vi "TDMS_EnsureFile.vi"(8 "error in (no error)":errorcluster, 11 "Logger_state":T1={"ref TDMS"=refnum, "File Path"=path "", "counter"=0, "Folder tmp"=path "/home/lvuser/lab9data/tmp", "folder ready"=path "/home/lvuser/lab9data/ready"}) -> (0 "error out":errorcluster, 3 "state out":T1)   [LabVIEW 2025]
uses:
  Logger_State.ctl
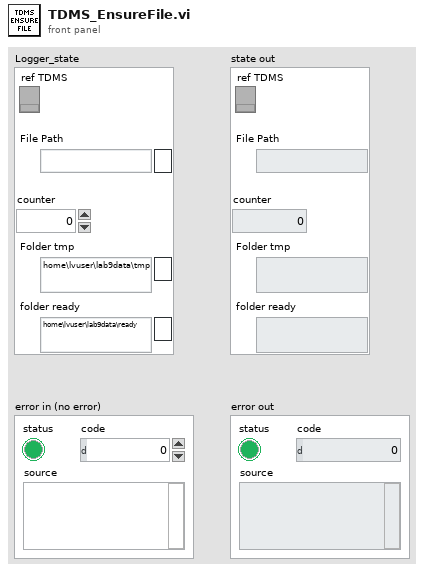
[diagram p1: front panel]
types:
  T1 = typedef "Logger_State.ctl" = cluster{"ref TDMS":refnum<k34>, "File Path":path, "counter":i32, "Folder tmp":path, "folder ready":path}
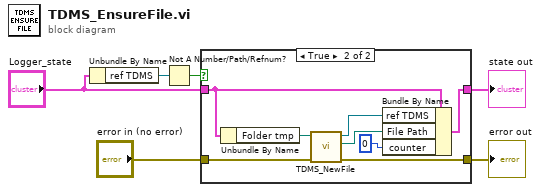
[diagram p0: block diagram]
diagram:
  n1 = Unbundle By Name("Logger_state") -> ("ref TDMS"=w1:refnum<k34>)
  n2 = Not A Number/Path/Refnum?(number/path/refnum=w1) -> (NaN/Path/Refnum?=w2:bool)
  n3 = case shown="True" w2 {
    tunnel: "Logger_state" -> [w7 w14]
    tunnel: "error in (no error)" -> [w8 w9]
    tunnel: [w8 w15] -> w5
    tunnel: [w7 w10] -> w6
    frame False {
    }
    frame True {
      n4 = Unbundle By Name(w14) -> ("Folder tmp"=w16:path)
      n5 = call "TDMS_NewFile.vi"("error in (no error)"=w9, "Folder tmp"=w16) -> ("error out"=w15:errorcluster, "Path"=w12:path, "Refnum out"=w13:refnum<k34>)  [unwired: 7 in]
      n6 = Bundle By Name(cluster=w14, "ref TDMS"=w13, "File Path"=w12, "counter"=0) -> (w10:T1)
    }
  }
  "error out" <- w5
  "state out" <- w6
